vi "temp_test.vi"(8 "error in (no error)":errorcluster) -> (0 "error out":errorcluster, 1 "temp txt_path":path, 2 "temp tdms_path B":path, 3 "temp_tdms":string, 5 "temp tdms_path A":path)   [LabVIEW 2018]
panel:
  out "temp_txt":string
  out "stripped path":path
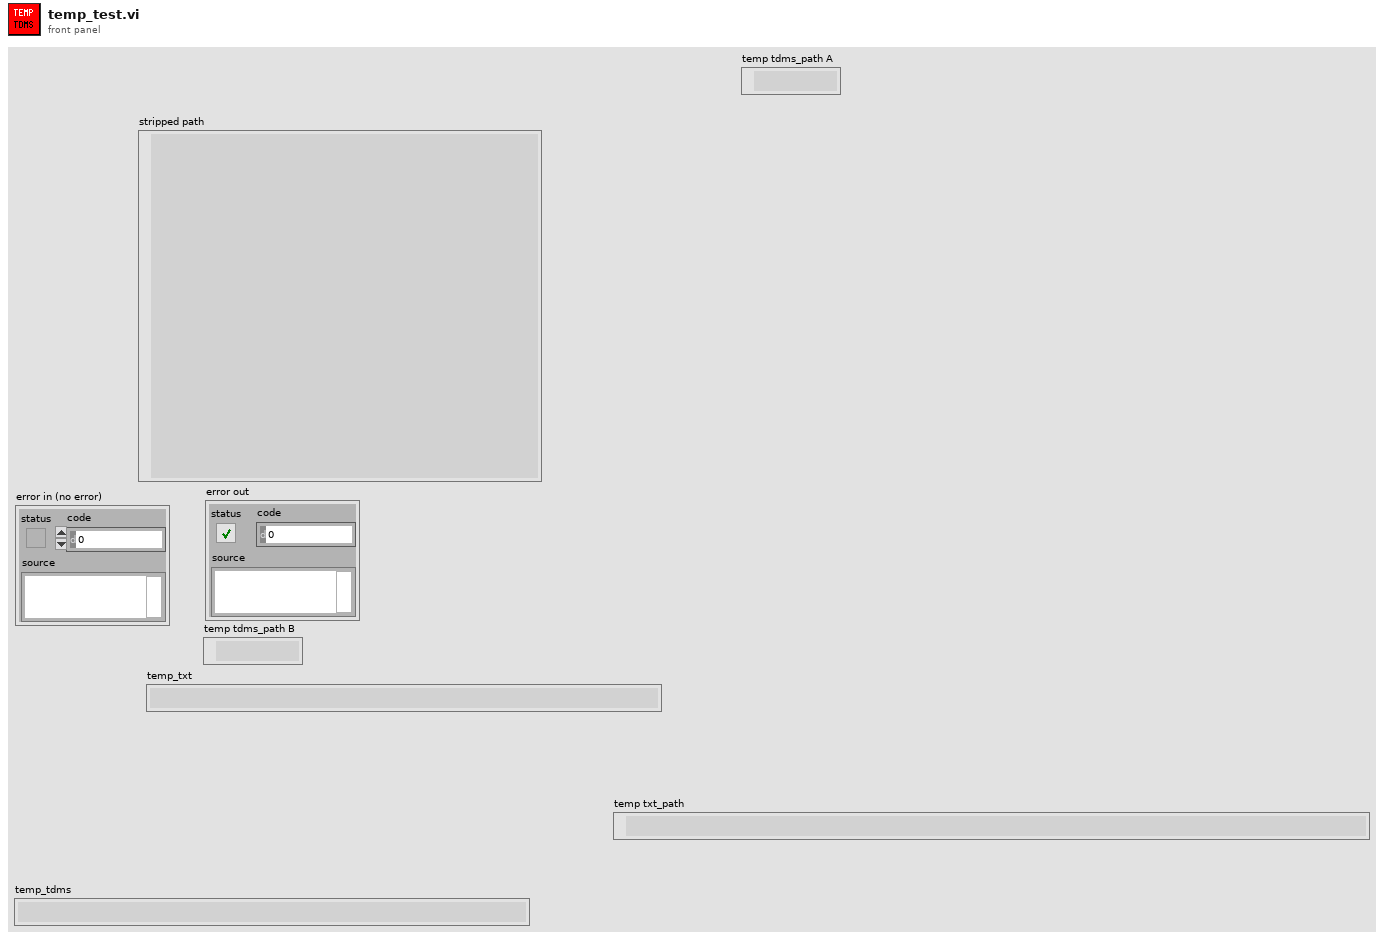
[diagram p1: front panel]
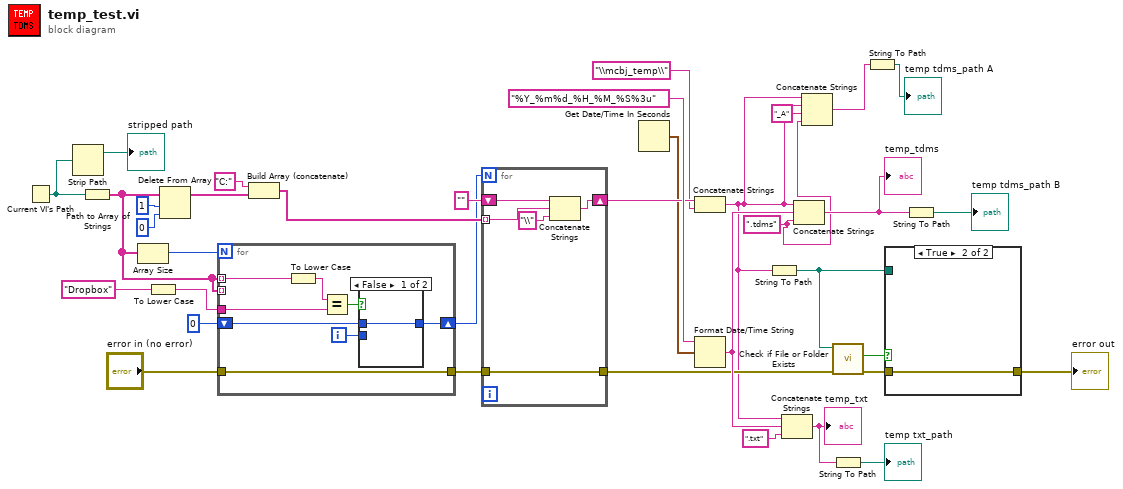
[diagram p0: block diagram]
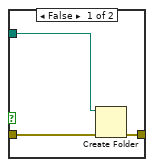
[diagram p2: hidden frame]
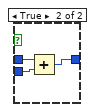
[diagram p3: hidden frame]
diagram:
  w3 = ".tdms" ("string")
  n1 = Current VI's Path() -> (path=w34:path)
  n2 = Strip Path(path=w34) -> (stripped path=→"stripped path":path)  [unwired: 1 out]
  n3 = Path to Array of Strings(0:w34) -> (2:w30:string[])  [unwired: 1 out]
  n4 = Array Size(array=w30) -> (size(s)=w33:i32)
  n5 = To Lower Case(string="Dropbox" ("正規表現")) -> (all lower case string=w31:string)
  n6 = Delete From Array(array=w30, length=1, index=0) -> (array with subset deleted=w27:string[])  [unwired: 1 out]
  n7 = for {
    N: w33 -> [_]
    tunnel: w30 -> [w43] mode=indexing
    tunnel: w31 -> [w44]
    tunnel: w30 -> [_] mode=indexing
    shift-right: [w39] -> w22
    shift-left: 0 -> [w38]
    tunnel: "error in (no error)" -> [w37]
    tunnel: [w37] -> w7
    i -> [w40]
    n8 = To Lower Case(string=w43) -> (all lower case string=w42:string)
    n9 = Equal?(x=w42, y=w44) -> (x = y?=w41:bool)
    n10 = case shown="False" w41 {
      tunnel: w40 -> [_ w48]
      tunnel: [w45 w47] -> w39
      tunnel: w38 -> [w45 w46]
      frame False {
      }
      frame True {
        n11 = Add(x=w46, y=w48) -> (x+y=w47:i32)
      }
    }
  }
  n12 = Build Array (concatenate)("C:" ("正規表現"), w27) -> (w25:string[])
  n13 = for {
    N: w22 -> [_]
    tunnel: w25 -> [w52] mode=indexing
    shift-right: [w53] -> w21
    shift-left: "" -> [w51]
    tunnel: w7 -> [w49]
    tunnel: [w49] -> w6
    n14 = Concatenate Strings(w51, w52, "\\" ("string")) -> (w53:string)
  }
  n15 = Get Date/Time In Seconds() -> (seconds since 1Jan1904=w19:timestamp)
  n16 = Concatenate Strings(w21, "\\mcbj_temp\\" ("string")) -> (w5:string)
  n17 = Format Date/Time String(time format string (%c)="%Y_%m%d_%H_%M_%S%3u" ("時間形式文字列（%c）"), seconds (now)=w19) -> (date/time string=w12:string)  [unwired: 1 in]
  n18 = String To Path(string=w5) -> (path=w18:path)
  n19 = Concatenate Strings(w5, w12, ".txt" ("string")) -> (w9:string)
  "temp_txt" <- w9
  n20 = Concatenate Strings(w5, w12, w3) -> (w14:string)
  "temp_tdms" <- w14
  n21 = Concatenate Strings(w5, w5, "_A" ("string"), w3) -> (w2:string)
  n22 = call <vilib>:"Check if File or Folder Exists.vi"("error in (no error)"=w6, "path"=w18) -> ("error out"=w16:errorcluster, "file or folder exists?"=w17:bool)  [unwired: 7 in, 1 out]
  n23 = String To Path(string=w9) -> (path=→"temp txt_path":path)
  n24 = String To Path(string=w2) -> (path=→"temp tdms_path A":path)
  n25 = case shown="True" w17 {
    tunnel: w18 -> [w56 _]
    tunnel: w16 -> [w55 w57]
    tunnel: [w54 w57] -> w15
    frame False {
      n26 = Create Folder(path (use dialog)=w56, error in=w55) -> (error out=w54:errorcluster)  [unwired: 1 in, 2 out]
    }
    frame True {
    }
  }
  "error out" <- w15
  n27 = String To Path(string=w14) -> (path=→"temp tdms_path B":path)
